vi "Linker.Remove sub tests.vi"(10 "Linker.Read Info From File":T2(array[cluster]), 11 "Tests":path[](array[path])) -> (3 "Array":path[](array[path]))   [LabVIEW 2020, in "Caraya.lvlib" / "Test Runner.lvclass"]
uses:
  Test Runner/Test Runner.lvclass
  <vilib>/Utility/lvfile.llb/LVFileType.ctl
  <vilib>/Utility/lvfile.llb/NI_FileType.lvlib
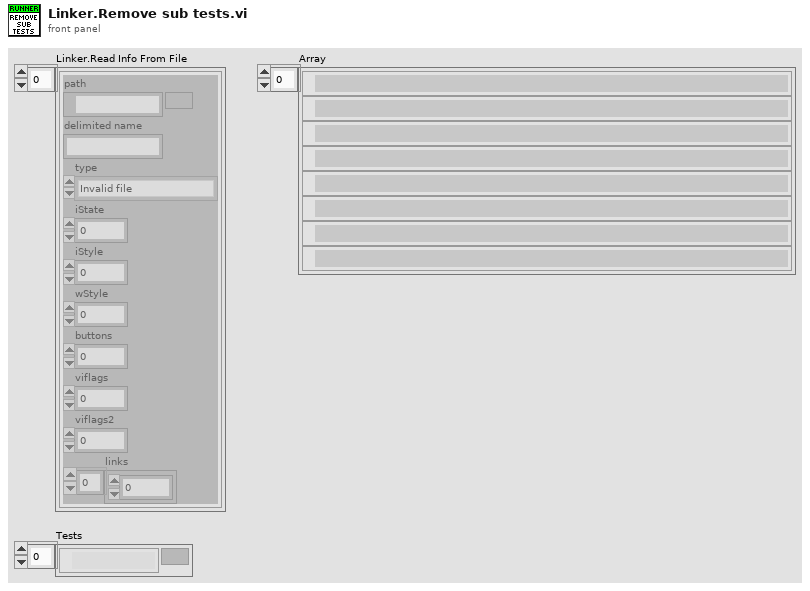
[diagram p1: front panel]
types:
  T1 = typedef "NI_FileType.lvlib/LVFileType.ctl" = enum32{"Invalid file", "Unknown type", "Instrument", "Control", "Polymorphic VI", "Project", "Library", "LVClass", "XControl", "XNode", "Shared library", ".NET assembly", "ActiveX interface", "CIN", "Run-time menu", "Palette menu", "Help file", "LLB", "XNode Edit Dependency", "Class Private Data Control", "Statechart", "MathScript .m file", "Ladder Diagram", "LVLibp", "XNode Build Dependency"}
  T2 = cluster{"path":path, "delimited name":string, "type":T1, "iState":u32, "iStyle":u16, "wStyle":u16, "buttons":u16, "viflags":u32, "viflags2":u32, "links":u32[]}[]
  T3 = cluster{"path":path, "delimited name":string, "type":T1, "iState":u32, "iStyle":u16, "wStyle":u16, "buttons":u16, "viflags":u32, "viflags2":u32, "links":u32[]}
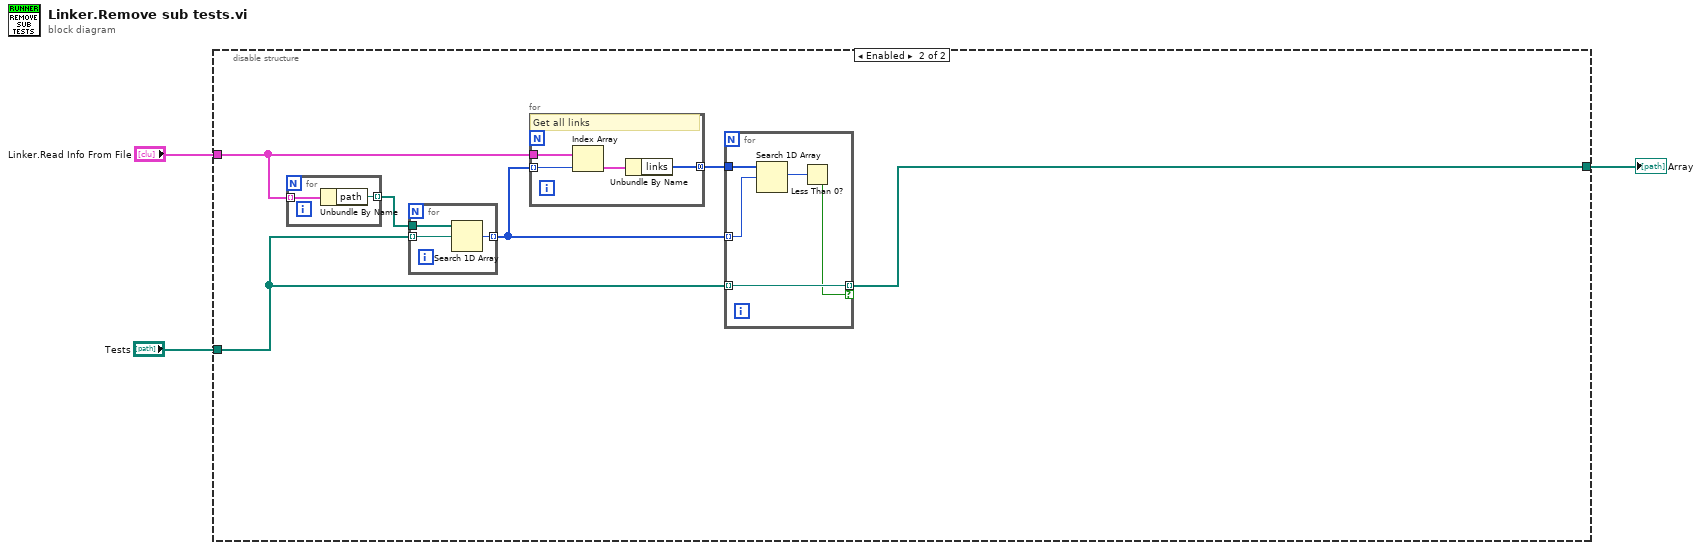
[diagram p0: block diagram]
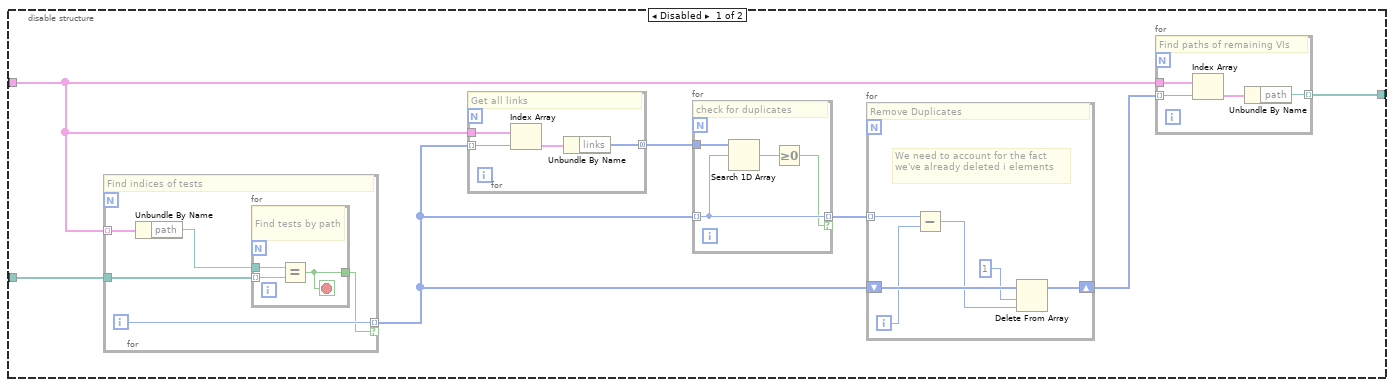
[diagram p2: hidden frame]
diagram:
  n1 = disable-structure shown="Enabled" {
    disable-tunnel: [w10 w37] -> w3
    disable-tunnel: "Linker.Read Info From File" -> [w9 w39]
    disable-tunnel: "Tests" -> [w4 w38]
    frame Disabled {
      n2 = for {
        tunnel: w9 -> [w33] mode=indexing
        tunnel: w4 -> [w31]
        tunnel: [w30] -> w7 mode=indexing if=w29
        i -> [w30]
        # "Find indices of tests"
        n3 = Unbundle By Name(w33) -> ("path"=w32:path)
        n4 = for {
          tunnel: w32 -> [w36]
          tunnel: w31 -> [w35] mode=indexing
          tunnel: [w34] -> w29
          stop <- w34 stop-if-true
          # "Find tests by path"
          n5 = Equal?(x=w36, y=w35) -> (x = y?=w34:bool)
        }
      }
      n6 = for {
        tunnel: w7 -> [w27] mode=indexing
        tunnel: w9 -> [w28]
        tunnel: [w25] -> w5 mode=concatenating
        # "Get all links"
        n7 = Index Array(array=w28, index=w27) -> (element=w26:T3)
        n8 = Unbundle By Name(w26) -> ("links"=w25:u32[])
      }
      n9 = for {
        tunnel: w5 -> [w24]
        tunnel: w7 -> [w22] mode=indexing
        tunnel: [w22] -> w6 mode=indexing if=w21
        # "check for duplicates"
        n10 = Search 1D Array(1D array=w24, element=w22) -> (index of element=w23:i32)  [unwired: 1 in]
        n11 = Greater Or Equal To 0?(x=w23) -> (x >= 0?=w21:bool)
      }
      n12 = for {
        tunnel: w6 -> [w19] mode=indexing
        shift-right: [w15] -> w8
        shift-left: w7 -> [w20]
        i -> [w18]
        # "We need to account for the fact we've already deleted i elements"
        # "Remove Duplicates"
        n13 = Subtract(x=w19, y=w18) -> (x-y=w17:i32)
        n14 = Delete From Array(array=w20, length=1, index=w17) -> (array with subset deleted=w15:i32[])  [unwired: 1 out]
      }
      n15 = for {
        tunnel: w8 -> [w13] mode=indexing
        tunnel: w9 -> [w14]
        tunnel: [w11] -> w10 mode=indexing
        # "Find paths of remaining VIs"
        n16 = Index Array(array=w14, index=w13) -> (element=w12:T3)
        n17 = Unbundle By Name(w12) -> ("path"=w11:path)
      }
    }
    frame Enabled {
      n18 = for {
        tunnel: w39 -> [w56] mode=indexing
        tunnel: [w55] -> w42 mode=indexing
        n19 = Unbundle By Name(w56) -> ("path"=w55:path)
      }
      n20 = for {
        tunnel: w42 -> [w54]
        tunnel: w38 -> [w53] mode=indexing
        tunnel: [w52] -> w40 mode=indexing
        n21 = Search 1D Array(1D array=w54, element=w53) -> (index of element=w52:i32)  [unwired: 1 in]
      }
      n22 = for {
        tunnel: w40 -> [w50] mode=indexing
        tunnel: w39 -> [w51]
        tunnel: [w48] -> w41 mode=concatenating
        # "Get all links"
        n23 = Index Array(array=w51, index=w50) -> (element=w49:T3)
        n24 = Unbundle By Name(w49) -> ("links"=w48:u32[])
      }
      n25 = for {
        tunnel: w41 -> [w47]
        tunnel: w40 -> [w46] mode=indexing
        tunnel: w38 -> [w44] mode=indexing
        tunnel: [w44] -> w37 mode=indexing if=w43
        n26 = Search 1D Array(1D array=w47, element=w46) -> (index of element=w45:i32)  [unwired: 1 in]
        n27 = Less Than 0?(x=w45) -> (x < 0?=w43:bool)
      }
    }
  }
  "Array" <- w3
